vi "Read Port.vi"(8 "error in (no error)":errorcluster, 11 "Modbus_TCP in":refnum<class "Modbus_TCP.lvclass">) -> (0 "error out":errorcluster, 2 "port (502)":u16=502, 3 "Modbus_TCP out":refnum<class "Modbus_TCP.lvclass">)   [LabVIEW 2021, in "Modbus_TCP.lvclass"]
uses:
  Modbus_TCP.lvclass
  Modbus_TCP.lvclass/Modbus_TCP.ctl
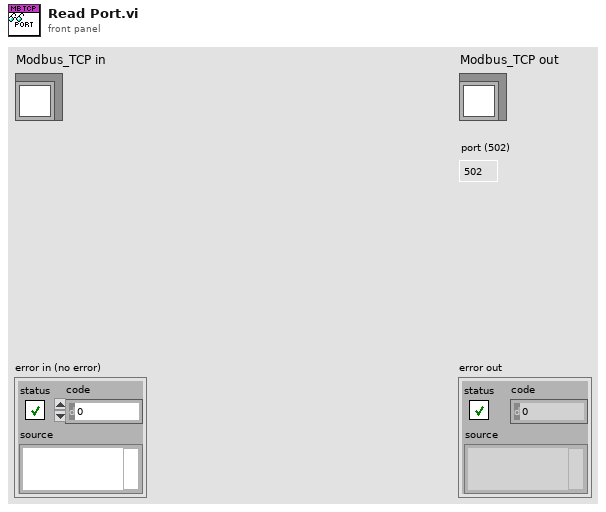
[diagram p1: front panel]
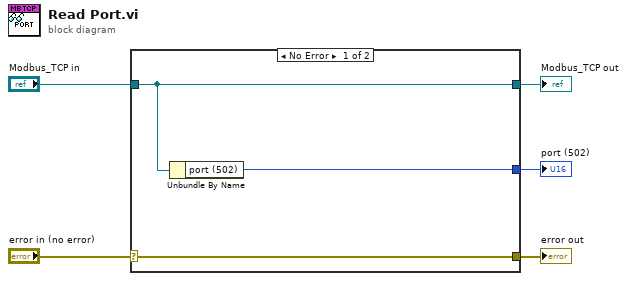
[diagram p0: block diagram]
diagram:
  n1 = case shown="No Error" "error in (no error)" {
    selector: "error in (no error)" -> [w8 w9]
    tunnel: [w8 w9] -> w4
    tunnel: [w7 w10] -> w2
    tunnel: "Modbus_TCP in" -> [w7 w10]
    tunnel: [w6 _] -> w1
    frame No Error {
      n2 = Unbundle By Name(w7) -> ("port (502)"=w6:u16)
    }
    frame Error {
    }
  }
  "error out" <- w4
  "Modbus_TCP out" <- w2
  "port (502)" <- w1
